vi "Executor_Begin_Group.vi"(8 "error in (no error)":errorcluster={"status"=FALSE, "code"=0, "source"="\"\""}, 10 "RunContext":string, 11 "GroupDefinition":string) -> (0 "error out":errorcluster={"status"=FALSE, "code"=0, "source"="\"\""}, 2 "status ok":bool, 3 "GroupContext":string)   [LabVIEW 2026]
doc: "INTENT: Initialize group-level execution. LOGIC: Create branch contexts and cycle counters; register declared resource sets."
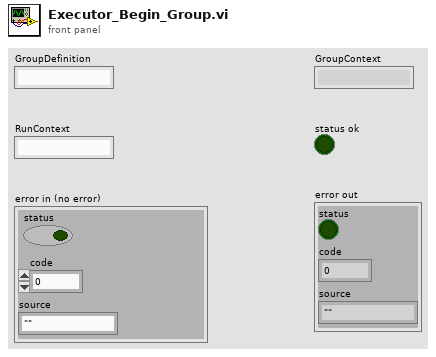
[diagram p1: front panel]
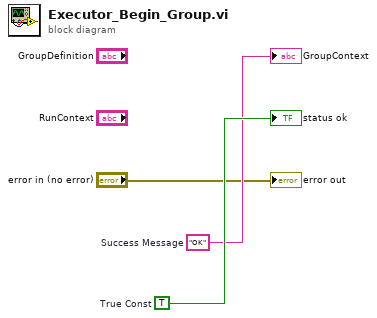
[diagram p0: block diagram]
diagram:
  w3 = TRUE  # True Const
  w2 = "OK"  # Success Message
  "GroupContext" <- w2
  "status ok" <- w3
  "error out" <- "error in (no error)"
